vi "RT_Flow_PID_Loop.vi"(8 "error in (no error)":errorcluster={"status"=FALSE, "code"=0, "source"="\"\""}, 10 "flow PV":string, 11 "Flow SP":string) -> (0 "error out":errorcluster={"status"=FALSE, "code"=0, "source"="\"\""}, 2 "status ok":bool, 3 "VFD speed request":string)   [LabVIEW 2026]
doc: "INTENT: Regulate hydraulic flow using VFD. LOGIC: Mode management; validate PV, compute PID, clamp limits, apply anti-windup and report saturation."
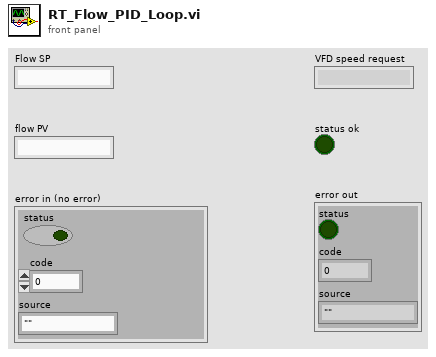
[diagram p1: front panel]
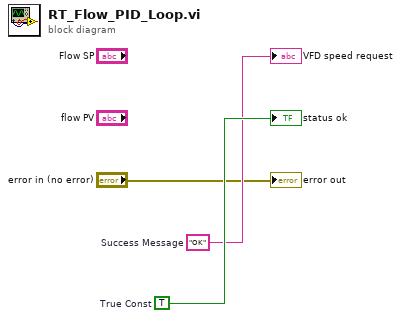
[diagram p0: block diagram]
diagram:
  w3 = TRUE  # True Const
  w2 = "OK"  # Success Message
  "VFD speed request" <- w2
  "status ok" <- w3
  "error out" <- "error in (no error)"
